vi "Native Toast Example.vi"(8 "error in":errorcluster) -> (0 "error out":errorcluster, 3 "Toast XML":string)   [LabVIEW 2026]
doc: "Native interop example using Toast Native.lvlib directly. Builds a toast with text, activation arguments, a text input and a button, reads XML, displays the toast and closes its acquired button, content and builder references. This example does not register an activation callback. Prefer Build Toast With Classes.vi for the public API and reply handling."
uses:
  Toast Native/Toast Native.lvlib
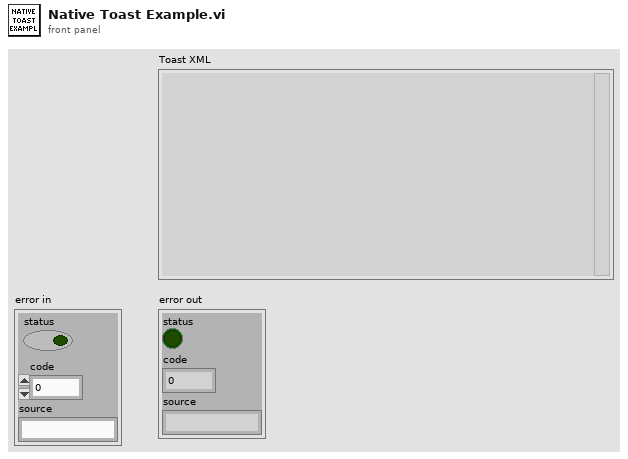
[diagram p1: front panel]
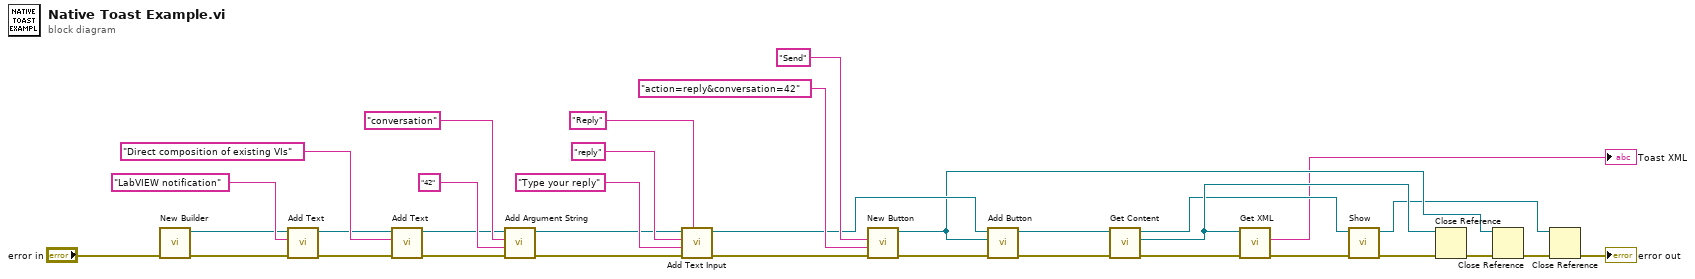
[diagram p0: block diagram]
diagram:
  n1 = call "New Builder.vi"("error in (no error)"="error in") -> ("error out"=w13:errorcluster, "new reference"=w11:refnum<k24>)  [unwired: 9 in]
  n2 = call "Add Text.vi"("error in (no error)"=w13, "text"="LabVIEW notification", "reference"=w11) -> ("error out"=w15:errorcluster, "reference out"=w10:refnum<k24>)  [unwired: 7 in]
  n3 = call "Add Text.vi"("error in (no error)"=w15, "text"="Direct composition of existing VIs", "reference"=w10) -> ("error out"=w17:errorcluster, "reference out"=w9:refnum<k24>)  [unwired: 7 in]
  n4 = call "Add Argument String.vi"("error in (no error)"=w17, "value"="42", "key"="conversation", "reference"=w9) -> ("error out"=w20:errorcluster, "reference out"=w8:refnum<k24>)  [unwired: 6 in]
  n5 = call "Add Text Input.vi"("title"="Reply", "error in (no error)"=w20, "placeHolderContent"="Type your reply", "id"="reply", "reference"=w8) -> ("error out"=w24:errorcluster, "reference out"=w7:refnum<k24>)  [unwired: 5 in]
  n6 = call "New Button.vi"("error in (no error)"=w24, "arguments"="action=reply&conversation=42", "content"="Send") -> ("error out"=w27:errorcluster, "new reference"=w6:refnum<k24>)  [unwired: 7 in]
  n7 = call "Add Button.vi"("error in (no error)"=w27, "button"=w6, "reference"=w7) -> ("error out"=w28:errorcluster, "reference out"=w5:refnum<k24>)  [unwired: 7 in]
  n8 = call "Get Content.vi"("error in (no error)"=w28, "reference"=w5) -> ("error out"=w29:errorcluster, "Content"=w4:refnum<k24>, "reference out"=w3:refnum<k24>)  [unwired: 7 in]
  n9 = call "Get XML.vi"("error in (no error)"=w29, "reference"=w4) -> ("error out"=w30:errorcluster, "GetContent"=→"Toast XML":string)  [unwired: 7 in, 1 out]
  n10 = call "Show.vi"("error in (no error)"=w30, "reference"=w3) -> ("error out"=w31:errorcluster, "reference out"=w2:refnum<k24>)  [unwired: 8 in]
  n11 = Close Reference(reference=w4, error in (no error)=w31) -> (error out=w32:errorcluster)
  n12 = Close Reference(reference=w6, error in (no error)=w32) -> (error out=w33:errorcluster)
  n13 = Close Reference(reference=w2, error in (no error)=w33) -> (error out=→"error out":errorcluster)
